vi "Convert to MB Address Cluster.vi"(10 "String":string, 11 "Device Settings":T1) -> (3 "Modbus Input/output cluster":T2)   [LabVIEW 2021]
uses:
  Modbus Address Cluster.ctl
  TypeDefs/Device Settings.ctl
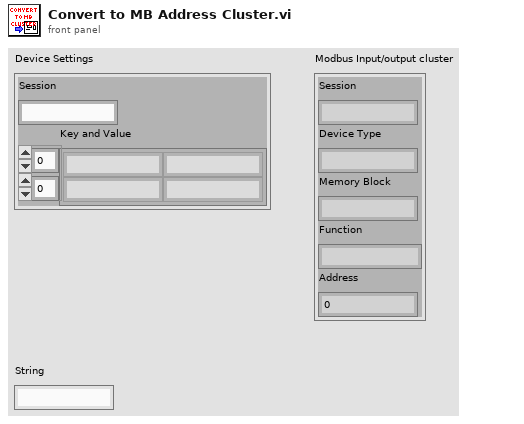
[diagram p1: front panel]
types:
  T1 = typedef "Device Settings.ctl" = cluster{"Session":string, "Key and Value":string[][]}
  T2 = typedef "Modbus Address Cluster.ctl" = cluster{"Session":string, "Device Type":string, "Memory Block":string, "Function":string, "Address":u16}
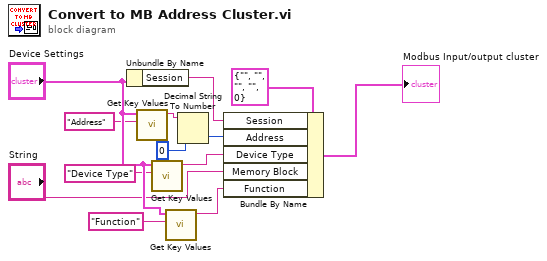
[diagram p0: block diagram]
diagram:
  n1 = Unbundle By Name("Device Settings") -> ("Session"=w2:string)
  n2 = call "Get Key Values.vi"("Search Key"="Address" ("key"), "Configure Cluster"="Device Settings") -> ("value"=w3:string)  [unwired: 8 in, 1 out]
  n3 = call "Get Key Values.vi"("Search Key"="Device Type" ("key"), "Configure Cluster"="Device Settings") -> ("value"=w10:string)  [unwired: 8 in, 1 out]
  n4 = call "Get Key Values.vi"("Search Key"="Function" ("key"), "Configure Cluster"="Device Settings") -> ("value"=w8:string)  [unwired: 8 in, 1 out]
  n5 = Decimal String To Number(string=w3, default (0L)=u16 0 ("default (0 I32)")) -> (number=w6:u16)  [unwired: 1 in, 1 out]
  n6 = Bundle By Name(cluster=T2 {"Session"="", "Device Type"="", "Memory Block"="", "Function"="", "Address"=0}, "Session"=w2, "Address"=w6, "Device Type"=w10, "Memory Block"="String", "Function"=w8) -> (→"Modbus Input/output cluster":T2)
